vi "Transport_Init.vi"(8 "error in (no error)":errorcluster={"status"=FALSE, "code"=0, "source"="\"\""}, 10 "target endpoint":string, 11 "Connection configuration":string) -> (0 "error out":errorcluster={"status"=FALSE, "code"=0, "source"="\"\""}, 2 "status ok":bool, 3 "Transport references and status":string)   [LabVIEW 2026]
doc: "INTENT: Construct Host/target communication channels. LOGIC: Open command-down, reply-up, event-up and heartbeat channels according to deployment profile."
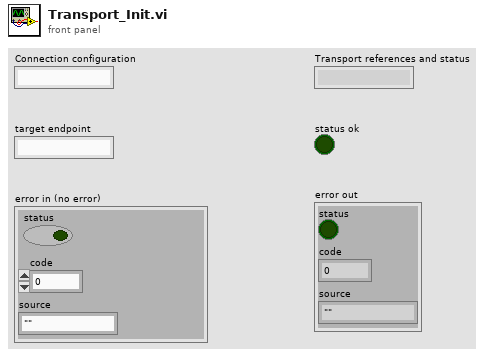
[diagram p1: front panel]
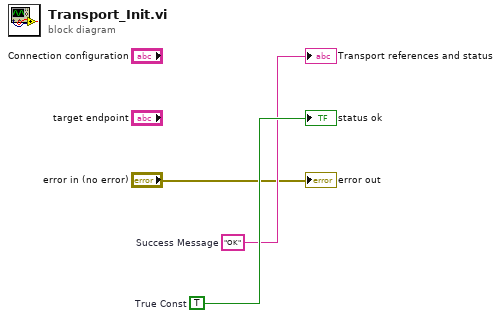
[diagram p0: block diagram]
diagram:
  w3 = TRUE  # True Const
  w2 = "OK"  # Success Message
  "Transport references and status" <- w2
  "status ok" <- w3
  "error out" <- "error in (no error)"
